vi "Add to Tree.vi"(8 "error in":errorcluster, 11 "Data in":T1={"PeekVI Reference"=refnum, "SubPanel"=refnum, "Peek Stack Tree Ref"=refnum, "Open Button Ref"=refnum, "Top VI"=refnum, "Active VI"=refnum, "Stack"=[], "Last FP State"=enum."Standard"}) -> (0 "error out":errorcluster, 3 "Data out":T1={"PeekVI Reference"=refnum, "SubPanel"=refnum, "Peek Stack Tree Ref"=refnum, "Open Button Ref"=refnum, "Top VI"=refnum, "Active VI"=refnum, "Stack"=[], "Last FP State"=enum."Standard"})   [LabVIEW 2020, in "Peek Window.lvlib"]
uses:
  Peek Window.lvlib
  MHL Data Cluster.ctl
  VI Types/Standard VI Type/Standard VI Type.lvclass
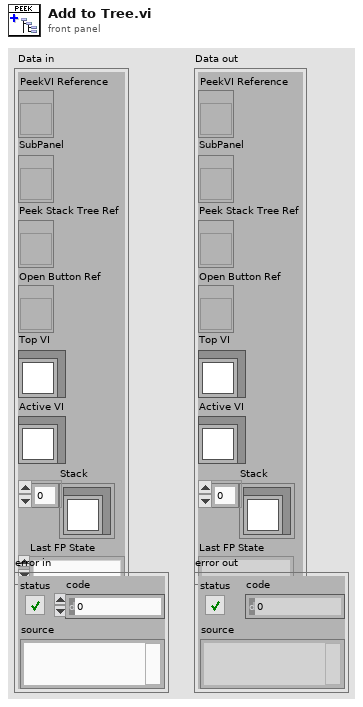
[diagram p1: front panel]
types:
  T1 = typedef "Peek Window.lvlib/MHL Data Cluster.ctl" = cluster{"PeekVI Reference":refnum<vi>, "SubPanel":refnum<vi>, "Peek Stack Tree Ref":refnum<vi>, "Open Button Ref":refnum<vi>, "Top VI":refnum<class "Standard VI Type.lvclass">, "Active VI":refnum<class "Standard VI Type.lvclass">, "Stack":refnum<class "Standard VI Type.lvclass">[], "Last FP State":enum32{"Invalid", "Standard", "Closed", "Hidden", "Minimized", "Maximized"}}
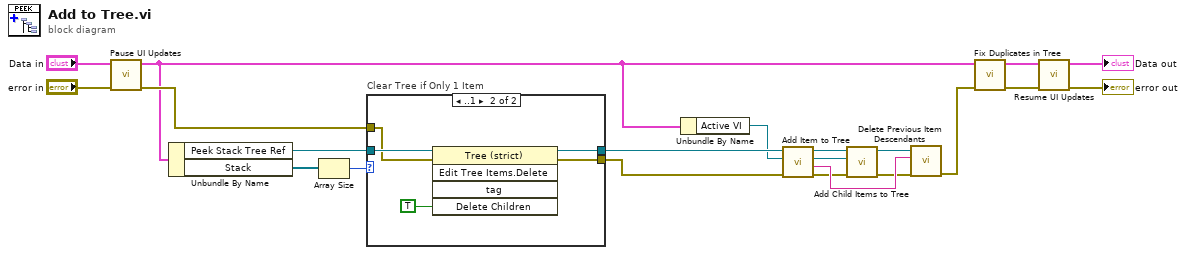
[diagram p0: block diagram]
diagram:
  n1 = call "Pause UI Updates.vi"("error in"="error in", "Module Data"="Data in") -> ("error out"=w16:errorcluster, "Module Data"=w4:T1)  [unwired: 8 in]
  n2 = Unbundle By Name(w4) -> ("Peek Stack Tree Ref"=w21:refnum<vi>, "Stack"=w20:refnum<class "Standard VI Type.lvclass">[])
  n3 = Array Size(array=w20) -> (size(s)=w19:i32)
  n4 = case "Clear Tree if Only 1 Item" shown="..1" w19 {
    tunnel: w21 -> [w22 w28]
    tunnel: w16 -> [w23 w26]
    tunnel: [w23 w25] -> w12
    tunnel: [w22 w24] -> w5
    frame Default {
      # "Multiple items in call chain, add new VI to end of tree"
    }
    frame ..1 {
      # "Only one item in call chain, delete current tree and add single item"
      n5 = invoke class="Tree (strict)" method="Edit Tree Items.Delete"(reference=w28, error in=w26, "Delete Children"=TRUE ("Delete Children?")) -> (reference out=w24:refnum<vi>, error out=w25:errorcluster)  [unwired: 2 in, 3 out]
    }
  }
  n6 = Unbundle By Name(w4) -> ("Active VI"=w3:refnum<class "Standard VI Type.lvclass">)
  n7 = call-dynamic "Add Item to Tree.vi"("error in (no error)"=w12, "Standard VI Type in"=w3, "Tree Ref in"=w5) -> ("error out"=w6:errorcluster, "Added Tag"=w11:string, "Standard VI Type out"=w7:refnum<class "Standard VI Type.lvclass">, "Tree Ref out"=w8:refnum<vi>)  [unwired: 5 in]
  n8 = call-dynamic "Add Child Items to Tree.vi"("error in (no error)"=w6, "Standard VI Type in"=w7, "Tree Ref in"=w8) -> ("error out"=w9:errorcluster, "Tree Ref out"=w10:refnum<vi>)  [unwired: 6 in, 1 out]
  n9 = call "Delete Previous Item Descendants.vi"("error in (no error)"=w9, "Edit Tree Items:Add Item to End"=w11, "TreeControl in"=w10) -> ("error out"=w2:errorcluster)  [unwired: 7 in, 1 out]
  n10 = call "Fix Duplicates in Tree.vi"("error in (no error)"=w2, "Data in"=w4) -> ("error out"=w1:errorcluster, "Data out"=w13:T1)  [unwired: 8 in]
  n11 = call "Resume UI Updates.vi"("error in"=w1, "Module Data"=w13) -> ("error out"=→"error out":errorcluster, "Module Data"=→"Data out":T1)  [unwired: 8 in]
